vi "Restart Discovery Service.vi"(8 "error in":errorcluster) -> (0 "error out":errorcluster)   [LabVIEW 2021, in "MeasurementServerTests.lvlib"]
uses:
  MeasurementServerTests.lvlib
  Runtime/Clients/Discovery V1/TypeDefs/gRPC Client Cache FGV Action.ctl
  Runtime/Clients/Discovery V1/NI Discovery V1 Client.lvlib
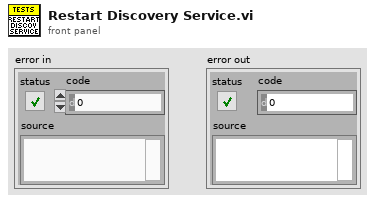
[diagram p1: front panel]
types:
  T1 = typedef "NI Discovery V1 Client.lvlib/gRPC Client Cache FGV Action.ctl" = enum16{"Get Client", "Recreate Client", "Destroy Client", "Update ClusterId"}
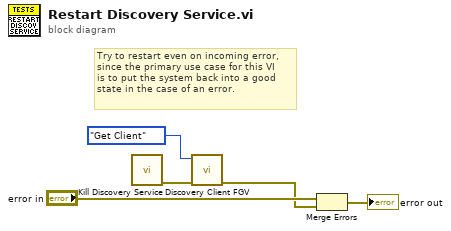
[diagram p0: block diagram]
diagram:
  # "Try to restart even on incoming error,\nsince the primary use case for this VI\nis to put the system back into a good \nstate in the case of an error."
  n1 = call "Kill Discovery Service.vi"() -> ("error out"=w2:errorcluster)  [unwired: 11 in]
  n2 = call "Discovery Client FGV.vi"("error in"=w2, "action"=gRPC_Client_Cache_FGV_Action."Get Client") -> ("error out"=w1:errorcluster)  [unwired: 6 in, 3 out]
  n3 = Merge Errors("error in", w1) -> (→"error out":errorcluster)
